vi "ComputeBlocks.vi"(7 "MD5":refnum<class "MD5.lvclass">, 10 "blocks queue":refnum<queue>) -> (2 "hash":u8[](array[numeric]) format="%02x")   [LabVIEW 2013, in "MD5.lvlib" / "MD5.lvclass"]
doc: "This VI contains the core of the MD5 algorithm."
uses:
  MD5.lvclass
  Data-vector.ctl
  K-Vector.vi
  S-Vector.vi
  F.vi
  G.vi
  H.vi
  I.vi
  T-Vector.vi
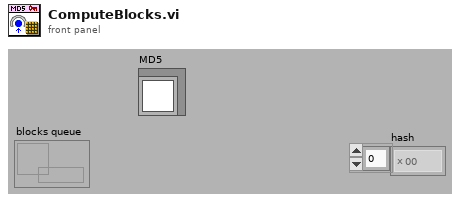
[diagram p1: front panel]
types:
  T1 = typedef "MD5.lvlib/MD5.lvclass/Data-vector.ctl" = cluster{"Data[ ]":u8[], "end":bool}
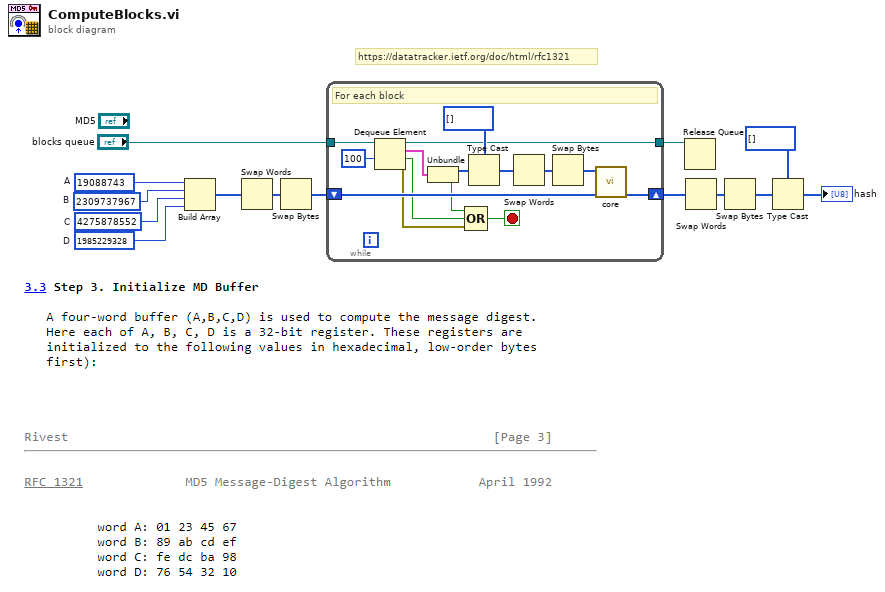
[diagram p0: block diagram]
diagram:
  w10 = u32 1985229328  # D
  w11 = u32 4275878552  # C
  w12 = u32 2309737967  # B
  w13 = u32 19088743  # A
  # "https://datatracker.ietf.org/doc/html/rfc1321"
  n1 = Build Array(w13, w12, w11, w10) -> (w8:u32[])
  n2 = Swap Words(1:w8) -> (0:w3:u32[])
  n3 = Swap Bytes(anything=w3) -> (byte swapped=w7:u32[])
  n4 = while {
    shift-right: [w28] -> w6
    shift-left: w7 -> [w29]
    tunnel: "blocks queue" -> [w27]
    tunnel: [w17] -> w1
    stop <- w18 stop-if-true
    # "For each block"
    n5 = Dequeue Element(queue=w27, timeout in ms (-1)=100) -> (queue out=w17:refnum<queue>, element=w26:T1, timed out?=w15:bool, error out=w24:errorcluster)  [unwired: 1 in]
    n6 = Unbundle(w26) -> ("Data[ ]"=w25:u8[], "end"=w23:bool)
    n7 = Compound Arithmetic op=OR(w23, w15, w24) -> (w18:bool)
    n8 = Type Cast(type=u32[] [] ("U32"), x=w25) -> (*(type *) &x=w19:u32[])
    n9 = Swap Words(1:w19) -> (0:w22:u32[])
    n10 = Swap Bytes(anything=w22) -> (byte swapped=w21:u32[])
    n11 = call "core.vi"("ABCD in"=w29, "M[ ]"=w21) -> ("ABCD out"=w28:u32[])  [unwired: 9 in]
  }
  n12 = Release Queue(queue=w1) -> ()  [unwired: 2 in, 3 out]
  n13 = Swap Words(1:w6) -> (0:w4:u32[])
  n14 = Swap Bytes(anything=w4) -> (byte swapped=w5:u32[])
  n15 = Type Cast(type=u8[] [], x=w5) -> (*(type *) &x=→"hash":u8[])
